vi "PicoScope3000aExampleStreamingAdvancedTrig.vi"() -> ()   [LabVIEW 2010]
doc: "This example demonstrates how to use the PicoScope Labview library to stream data from a PicoScope 5000 Series Device"
uses:
  ps3000a.dll
  ps3000aWrap.dll
  <vilib>/Waveform/DWDTOps.llb/DWDT Analog to Digital.vi
  PicoScope3000aLib/PicoScope3000aAnalogChannelSettings.ctl
  PicoScope3000aLib/PicoScope3000aDigitalChannelSettings.ctl
panel:
  in  "Pulse Width Qualifier Conditions":T1 {"Condition Logic" items=["AND", "OR", "XOR"]}
  in  "Digital Port  0":T2 {"Direction Channel 7" items=["Don't Care", "Low", "High", "Rising", "Falling"]; "Direction Channel 6" items=["Don't Care", "Low", "High", "Rising", "Falling"]; "Direction Channel 5" items=["Don't Care", "Low", "High", "Rising", "Falling"]; "Direction Channel 4" items=["Don't Care", "Low", "High", "Rising", "Falling"]; "Direction Channel 3" items=["Don't Care", "Low", "High", "Rising", "Falling"]; "Direction Channel 2" items=["Don't Care", "Low", "High", "Rising", "Falling"]; "Direction Channel 1" items=["Don't Care", "Low", "High", "Rising", "Falling"]; "Direction Channel 0" items=["Don't Care", "Low", "High", "Rising", "Falling"]}
  in  "Pulse Width Qualifier Settings":T3={"Direction"=2, "Lower Limit"=0, "Upper Limit"=0, "Pulse Width Type"=0} {"Pulse Width Type" items=["None", "Less Than", "Greater Than", "In Range", "Out of Range"]; "Direction" items=["Rising"=2, "Falling"=3]}
  in  "Auto Trigger (ms)":i32=1000
  in  "Trigger Conditions":T4 {"Condition Logic" items=["AND", "OR", "XOR"]}
  in  "Channel B Trigger Properties":T5={"thresholdUpper"=0, "thresholdUpperHysteresis"=1024, "thresholdLower"=0, "thresholdLowerHysteresis"=1024, "Threshold Mode"=0, "Direction"=2, "Available"=FALSE} {"Direction" items=["Above / Inside", "Below / Outside", "Rising / Enter", "Falling / Exit", "Rising or Falling / Enter or Exit", "Above Lower", "Below Lower", "Rising Lower", "Falling Lower", "Positive Runt", "Negative Runt"]; "Threshold Mode" items=["Level", "Window"]}
  in  "Channel A Trigger Properties":T5={"thresholdUpper"=0, "thresholdUpperHysteresis"=1024, "thresholdLower"=0, "thresholdLowerHysteresis"=1024, "Threshold Mode"=0, "Direction"=2, "Available"=FALSE} {"Direction" items=["Above / Inside", "Below / Outside", "Rising / Enter", "Falling / Exit", "Rising or Falling / Enter or Exit", "Above Lower", "Below Lower", "Rising Lower", "Falling Lower", "Positive Runt", "Negative Runt"]; "Threshold Mode" items=["Level", "Window"]}
  in  "Port 0 Settings":T6={"Enabled"=FALSE, "Logic Level"=9830} {"Logic Level" items=["1.5V TTL"=9830, "2.5V CMOS"=16383]}
  in  "Channel A Settings":T7={"Enabled"=TRUE, "Coupling"=1, "Range"=6, "Analogue Offset"=0.0, "Bandwidth Limit"=0} {"Bandwidth Limit" items=["Full", "20MHz"]; "Range" items=["10 mV", "20 mV", "50 mV", "100 mV", "200 mV", "500 mV", "1 V", "2 V", "5 V", "10 V", "20 V", "50 V ", "100 V"]; "Coupling" items=["AC", "DC"]}
  out "Analog Channels":T8(graph)
  out "Raw Sample Interval (sec)":dbl=1.0000000130088963e-06 format="%#.5p"
  out "Max ADC value":i16
  out "Chunk time":u32
  out "Elapsed time":dbl
  in  "Poll time (ms)":u32=10 min=1 max=1000 step=1
  in  "Data file":path=path "PicoScope3000aExampleStreaming ChA Data"
  out "size(s)":i32
  out "Queue depth":i32(graph)
  out "queue depth":i32
  in  "Buffer and Transfer Settings":T9={"startIndex"=0, "Samples"=1000000, "Down Sample Ratio"=1, "Down-Sample Mode"=0} {"Down-Sample Mode" items=["None"=0, "Aggregate"=1, "Decimate"=2, "Average"=4]; "Down Sample Ratio" step=1; "Samples" format="%_6p"}
  out "USB Powered":bool=TRUE
  out "USB 3.0 device on non-USB 3.0 Port":bool=TRUE
  out "TriggeredAt (In Buffer)":u32 format="%#.6p"
  out "TriggeredAt (Total samples)":u32 format="%#.6p"
  in  "Acquisition Settings":T10={"Auto Stop"=TRUE, "Desired Sample Interval"=1, "Pre-trigger Samples"=500000, "Post-trigger Samples"=500000, "Down-Sample Ratio"=1, "Down-Sample Mode"=0, "Time Units"=3} {"Time Units" items=["Nanoseconds (ns)"=2, "Microseconds (us)"=3, "Milliseconds (ms)"=4, "Seconds (s)"=5]; "Down-Sample Mode" items=["None"=0, "Aggregate"=1, "Decimate"=2, "Average"=4]; "Post-trigger Samples" format="%#.6p"; "Pre-trigger Samples" format="%#_6p"}
  out "Port 0":digitalwaveform(graph)={"t0"=timestamp(0 s since 1904-01-01), "dt"=1.0000000130088963e-06, "Y"={"transitions"=[], "data"=[]}}
  out "Triggered":bool
  out "DownSample Interval (sec)":dbl=1.0000000130088963e-06 format="%#.5p"
  out "Total Samples":u32 format="%#.6p"
  out "Auto Stopped":bool
  in  "Serial Number":string
  in  "Open Using Serial Number":bool
  out "Number of Samples per Capture":u32 format="%#.6p"
  in  "Apply  Settings":bool
  in  "stop":bool
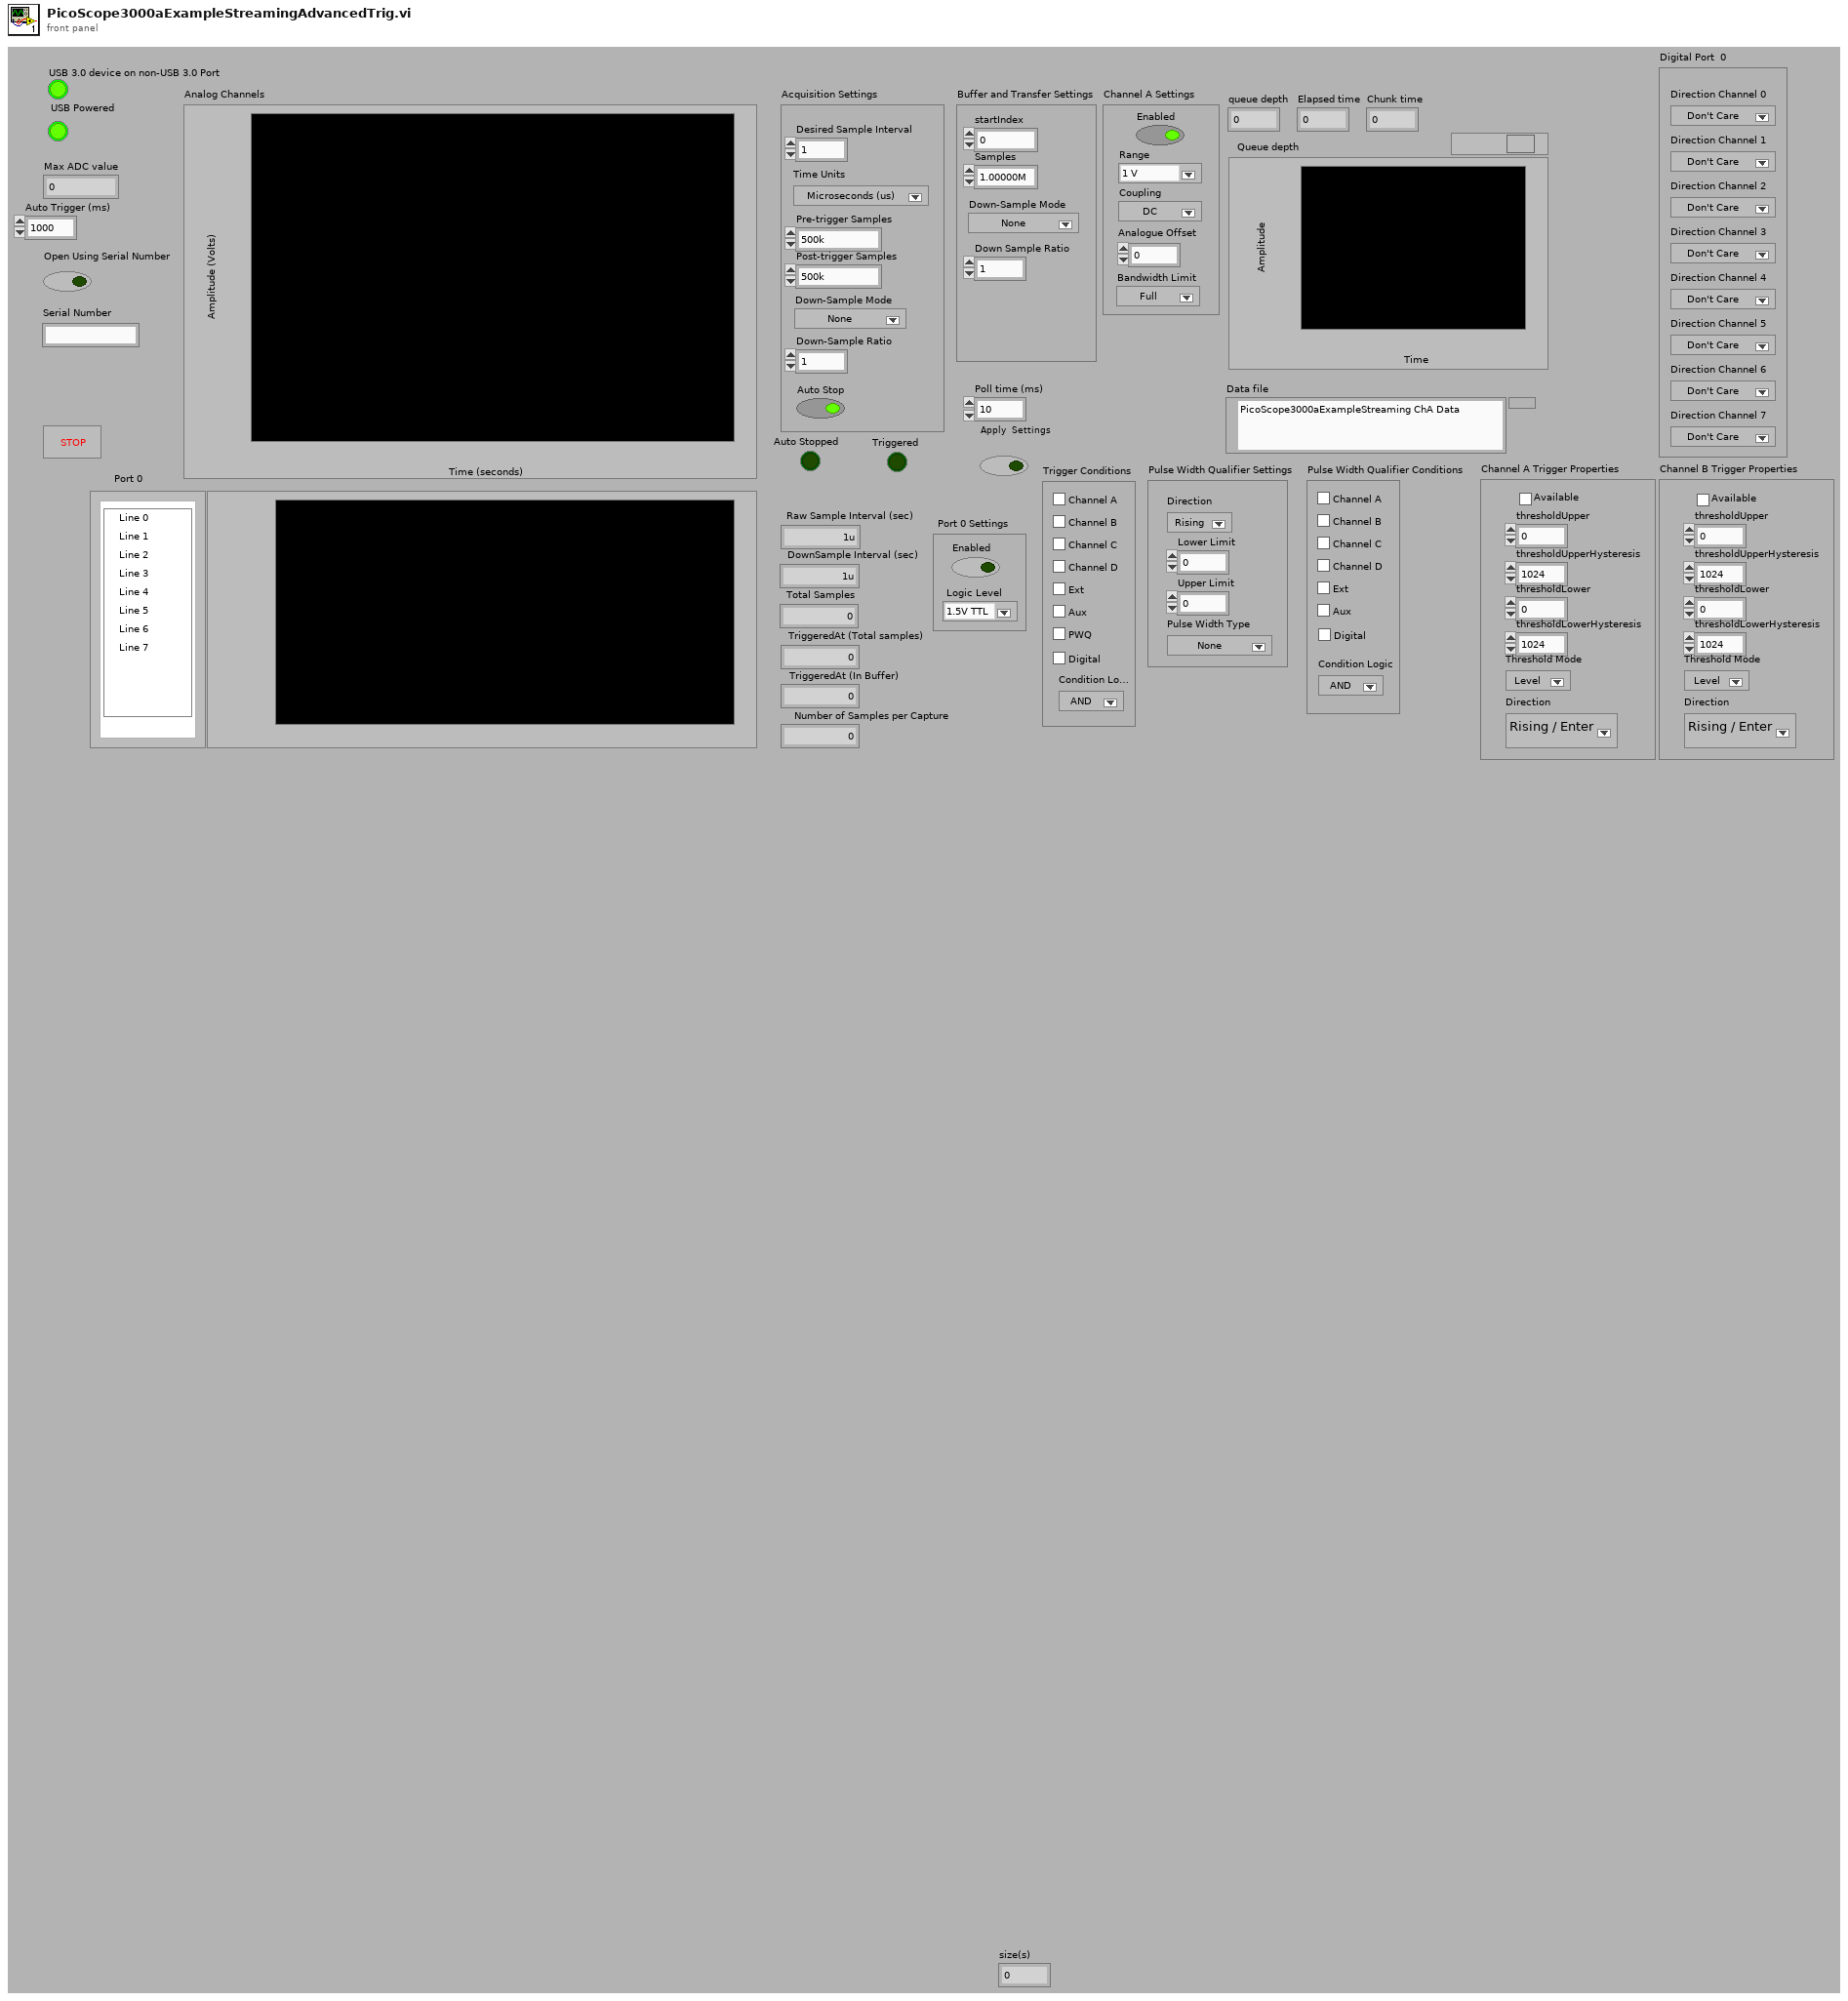
[diagram p1: front panel]
types:
  T1 = cluster{"Channel A":bool, "Channel B":bool, "Channel C":bool, "Channel D":bool, "Aux":bool, "Condition Logic":u16, "Ext":bool, "Digital":bool}
  T2 = cluster{"Direction Channel 0":u16, "Direction Channel 1":u16, "Direction Channel 2":u16, "Direction Channel 3":u16, "Direction Channel 4":u16, "Direction Channel 5":u16, "Direction Channel 6":u16, "Direction Channel 7":u16}
  T3 = cluster{"Direction":u32, "Lower Limit":u32, "Upper Limit":u32, "Pulse Width Type":u32}
  T4 = cluster{"Channel A":bool, "Channel B":bool, "Channel C":bool, "Channel D":bool, "Aux":bool, "PWQ":bool, "Condition Logic":u16, "Ext":bool, "Digital":bool}
  T5 = cluster{"thresholdUpper":i16, "thresholdUpperHysteresis":u16, "thresholdLower":i16, "thresholdLowerHysteresis":u16, "Threshold Mode":i32, "Direction":i32, "Available":bool}
  T6 = typedef "PicoScope3000aDigitalChannelSettings.ctl" = cluster{"Enabled":bool, "Logic Level":i16}
  T7 = typedef "PicoScope3000aAnalogChannelSettings.ctl" = cluster{"Enabled":bool, "Coupling":u32, "Range":u32, "Analogue Offset":sgl, "Bandwidth Limit":u32}
  T8 = cluster{i32, "DownSample Interval (sec)":dbl, "Data":dbl[]}
  T9 = cluster{"startIndex":u64, "Samples":u64, "Down Sample Ratio":u64, "Down-Sample Mode":u32}
  T10 = cluster{"Auto Stop":bool, "Desired Sample Interval":u32, "Pre-trigger Samples":u32, "Post-trigger Samples":u32, "Down-Sample Ratio":u32, "Down-Sample Mode":i32, "Time Units":u32}
  T11 = enum16{"open", "open or create", "create or replace", "create", "open (read-only)"}
  T12 = cluster{"Driver Version":string, "USB Version":string, "Hardware":string, "Variant":string, "Batch and Serial":string, "Cal Date":string, "Kernel Version":string, "Digital HW Version":string, "Analogue HW Version":string, "MSO":bool, "Number of channels":i16}
  T13 = cluster{"Channel A Buffer":i16[], "Channel B Buffer":i16[], "Channel C Buffer":i16[], "Channel D Buffer":i16[], "Channel E Buffer":i16[], "Channel F Buffer":i16[], "Channel G Buffer":i16[], "Channel H Buffer":i16[], "Port 0":i16[], "Port 1":i16[]}
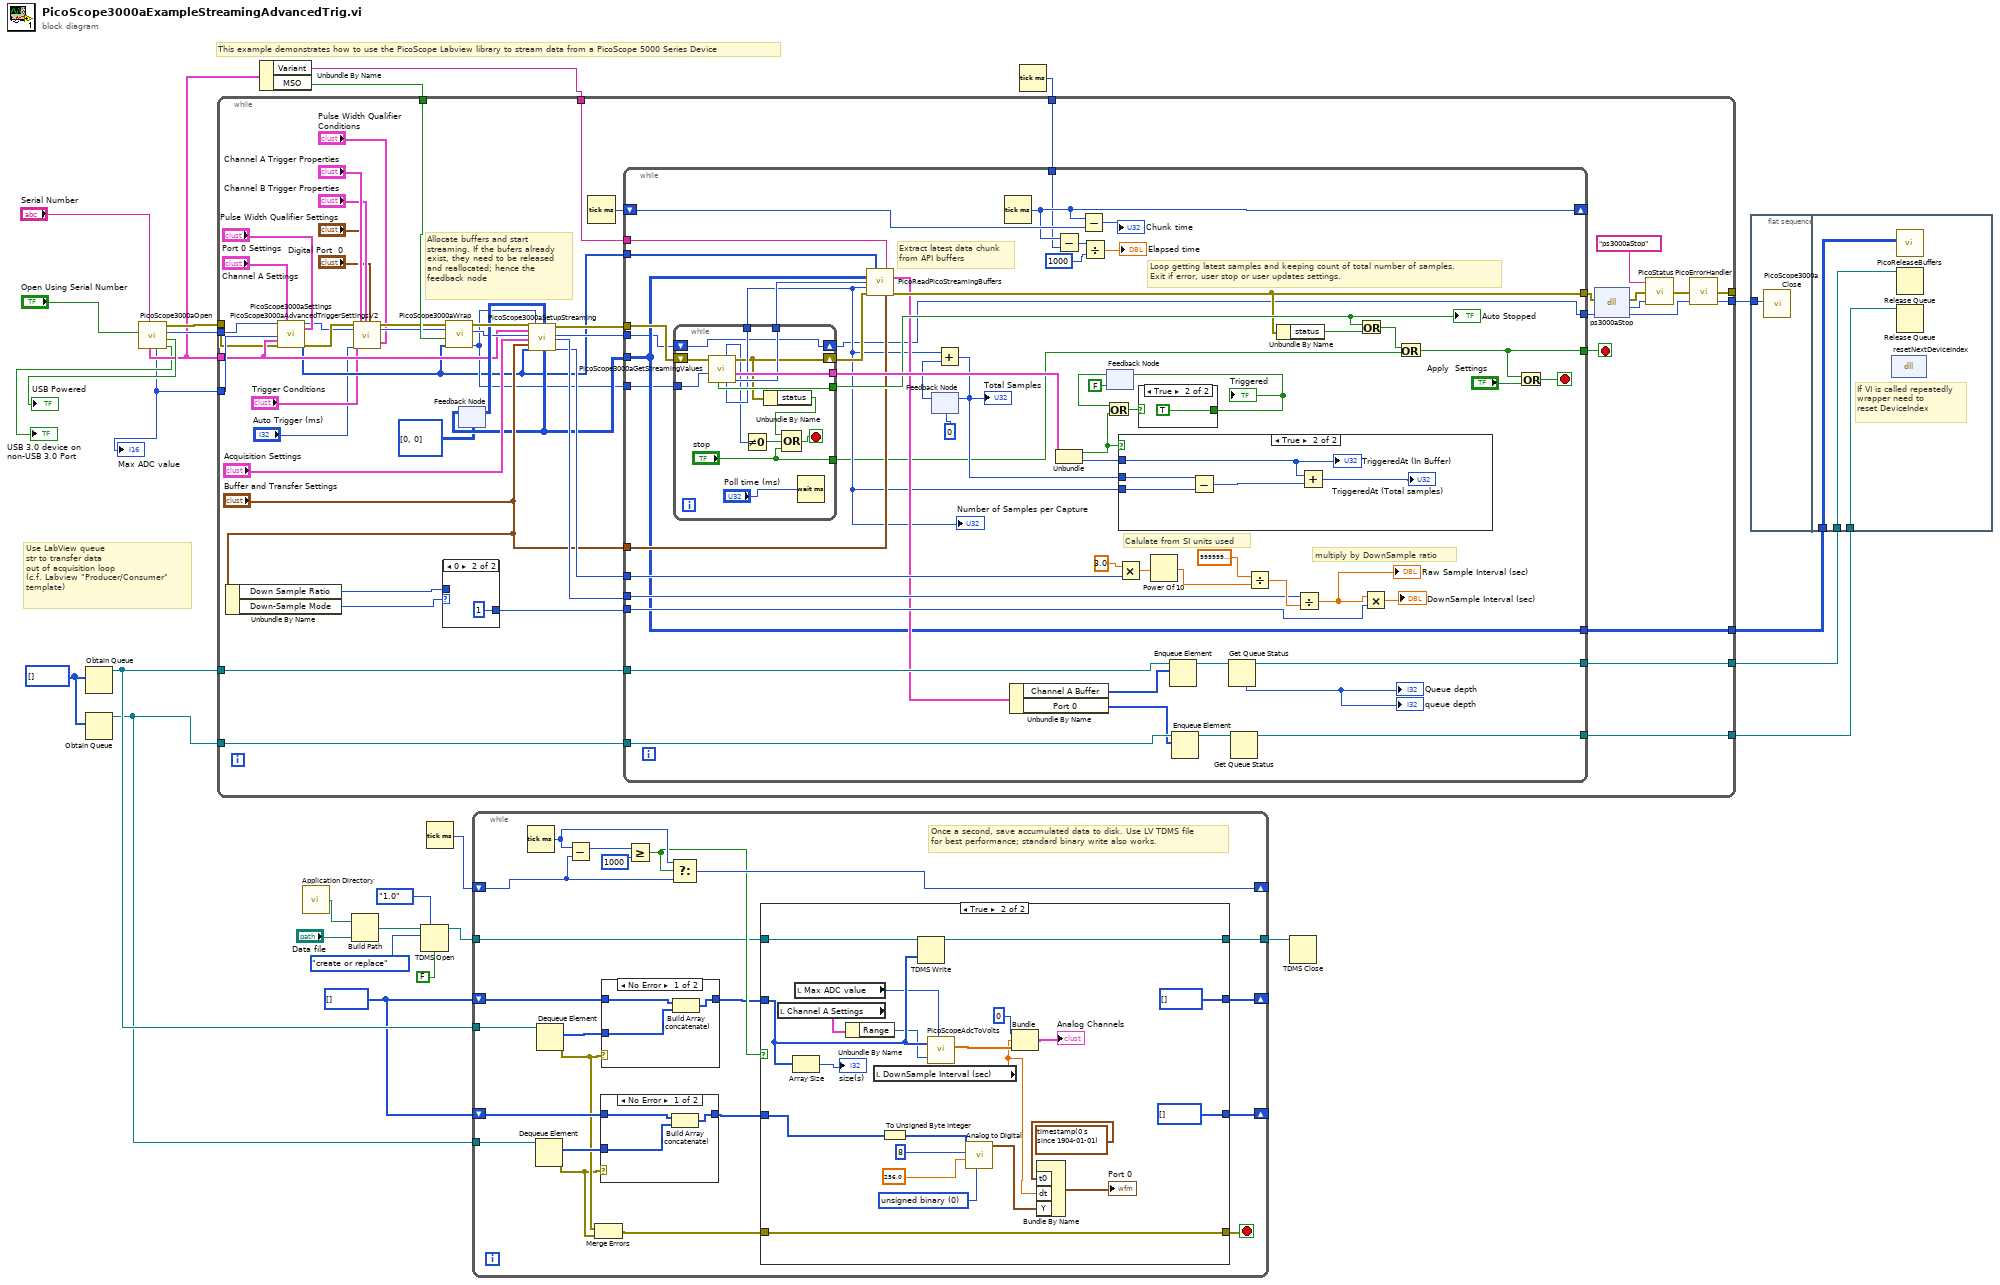
[diagram p0: block diagram]
diagram:
  w9 = i16[] [] ("History Data")
  w12 = i16[] [] ("History Data")
  # "Use LabView queue\nstr to transfer data\nout of acquisition loop\n(c.f. Labview \"Producer/Consumer\"\ntemplate)"
  # "This example demonstrates how to use the PicoScope Labview library to stream data from a PicoScope 5000 Series Device"
  n1 = Obtain Queue(element data type=w12) -> (queue out=w24:refnum<queue>)  [unwired: 4 in, 2 out]
  n2 = Obtain Queue(element data type=w12) -> (queue out=w10:refnum<queue>)  [unwired: 4 in, 2 out]
  n3 = call "PicoScope3000aOpen.vi"("Batch/Serial"="Serial Number", "Use Serial number"="Open Using Serial Number") -> ("USB 3.0 device on non-USB 3.0 Port"=→"USB 3.0 device on non-USB 3.0 Port":bool, "USB Powered"=→"USB Powered":bool, "handle"=w27:i16, "error out"=w28:errorcluster, "Max ADC value"=w1:i16, "Device Info"=w5:T12)  [unwired: 4 in]
  "Max ADC value" <- w1
  n4 = Unbundle By Name(w5) -> ("Variant"=w4:string, "MSO"=w3:bool)
  n5 = call <vilib>:"Application Directory.vi"() -> ("Application Directory"=w6:path)
  n6 = Build Path(base path=w6, name or relative path="Data file") -> (appended path=w7:path)
  n7 = TDMS Open(6:FALSE ("disable buffering? (T)"), 7:enum16{"1.0", "2.0"}."1.0" ("file format version (2.0)"), 10:T11."create or replace" ("operation (0:open)"), 11:w7) -> (3:w16:refnum<k34>)  [unwired: 2 in, 1 out]
  n8 = Tick Count (ms)() -> (millisecond timer value=w18:u32)
  n9 = while {
    tunnel: w24 -> [w49]
    shift-right: [w40] -> _
    shift-left: w9 -> [w48]
    shift-right: [w43] -> _
    shift-left: w18 -> [w44]
    tunnel: w16 -> [w39]
    tunnel: [w38] -> w15
    tunnel: w10 -> [w36]
    shift-right: [w33] -> _
    shift-left: w9 -> [w35]
    stop <- w30 stop-if-true
    # "Once a second, save accumulated data to disk. Use LV TDMS file\nfor best performance; standard binary write also works."
    n10 = Tick Count (ms)() -> (millisecond timer value=w45:u32)
    n11 = Dequeue Element(queue=w36) -> (element=w37:i16[], error out=w31:errorcluster)  [unwired: 2 in, 2 out]
    n12 = Dequeue Element(queue=w49) -> (element=w50:i16[], error out=w32:errorcluster)  [unwired: 2 in, 2 out]
    n13 = Subtract(x=w45, y=w44) -> (x-y=w47:u32)
    n14 = Merge Errors(w32, w31) -> (w29:errorcluster)
    n15 = case shown="No Error" w31 {
      tunnel: w35 -> [w53 w54]
      tunnel: [w52 w54] -> w34
      tunnel: w37 -> [w51 _]
      frame No Error {
        n16 = Build Array (concatenate)(w53, w51) -> (w52:i16[])
      }
      frame Error {
      }
    }
    n17 = case shown="No Error" w32 {
      tunnel: w48 -> [w83 w84]
      tunnel: [w82 w84] -> w41
      tunnel: w50 -> [w81 _]
      frame No Error {
        n18 = Build Array (concatenate)(w83, w81) -> (w82:i16[])
      }
      frame Error {
      }
    }
    n19 = Greater Or Equal?(x=w47, y=u32 1000) -> (x >= y?=w42:bool)
    n20 = Select(t=w45, s=w42, f=w44) -> (s? t:f=w43:u32)
    n21 = case shown="True" w42 {
      tunnel: w41 -> [w58 w76]
      tunnel: [w58 i16[] [] ("History Data")] -> w40
      tunnel: w39 -> [w57 w78]
      tunnel: [w57 w77] -> w38
      tunnel: w34 -> [w56 w63]
      tunnel: [w56 i16[] [] ("History Data")] -> w33
      tunnel: [w55 w59] -> w30
      tunnel: w29 -> [w55 w59]
      frame False {
      }
      frame True {
        w69 = u16 0 items=["unsigned binary", "offset binary", "2's complement"] ("data format (offset binary)")
        n22 = local read "Channel A Settings"() -> (w60:T7)
        n23 = Array Size(array=w76) -> (size(s)=→"size(s)":i32)
        n24 = local read "Max ADC value"() -> (w72:i16)
        n25 = Unbundle By Name(w60) -> ("Range"=w75:u32)
        n26 = local read "DownSample Interval (sec)"() -> (w64:dbl)
        n27 = To Unsigned Byte Integer(number=w63) -> (unsigned 8bit integer=w68:u8[])
        n28 = TDMS Write(0:w78, 9:w76) -> (4:w77:refnum<k34>)  [unwired: 4 in, 3 out]
        n29 = call "PicoScopeAdcToVolts.vi"("Max_adc"=w72, "Range Index"=w75, "Data"=w76) -> ("Data"=w73:dbl[])
        n30 = call-poly <vilib>:"Analog to Digital.vi"("data format (offset binary)"=w69, "full-scale range (pk-pk)"=256.0, "resolution (16 bit)"=8, "analog waveform"=w68) -> ("digital waveform"=w65:digitalwaveform)  [unwired: 4 in, 3 out]
        n31 = Bundle(0, "DownSample Interval (sec)"=w64, "Data"=w73) -> (→"Analog Channels":T8)  [unwired: 1 in]
        n32 = Bundle By Name("t0"=timestamp(0 s since 1904-01-01), "dt"=w64, "Y"=w65) -> (→"Port 0":digitalwaveform)  [unwired: 1 in]
      }
    }
  }
  n33 = Tick Count (ms)() -> (millisecond timer value=w23:u32)
  n34 = while {
    tunnel: [w131] -> w22
    tunnel: w28 -> [w98]
    tunnel: w27 -> [w97]
    tunnel: w5 -> [w100]
    tunnel: w1 -> [w103]
    tunnel: [w117] -> w20
    tunnel: w24 -> [w116]
    tunnel: [w115] -> w21
    tunnel: [w113] -> _
    tunnel: w23 -> [w111]
    tunnel: [w108] -> w11
    tunnel: w10 -> [w107]
    tunnel: w4 -> [w106]
    tunnel: w3 -> [w104]
    stop <- w135 stop-if-true
    # "Allocate buffers and start\nstreaming. If the bufers already\nexist, they need to be released\nand reallocated; hence the\nfeedback node"
    n35 = Unbundle By Name("Buffer and Transfer Settings") -> ("Down Sample Ratio"=w120:u64, "Down-Sample Mode"=w122:u32)
    n36 = call "PicoScope3000aSettings.vi"("handle in"=w97, "Channel A Settings"="Channel A Settings", "Port 0 Settings"="Port 0 Settings", "Max_adc"=w103, "Device Info"=w100, "error in"=w98) -> ("handle out"=w94:i16, "Enabled Array"=w96:i16[], "error out"=w95:errorcluster)  [unwired: 7 in]
    n37 = call "PicoScope3000aAdvancedTriggerSettingsV2.vi"("error in"=w95, "handle in"=w94, "Trigger Conditions"="Trigger Conditions", "Auto Trigger (ms)"="Auto Trigger (ms)", "Channel A Trigger Properties"="Channel A Trigger Properties", "Channel B Trigger Properties"="Channel B Trigger Properties", "Digital Port  0"="Digital Port  0", "Pulse Width Qualifier Conditions"="Pulse Width Qualifier Conditions", "Pulse Width Qualifier Settings"="Pulse Width Qualifier Settings") -> ("error out"=w93:errorcluster, "handle out"=w92:i16)  [unwired: 9 in]
    n38 = case shown="0" w122 {
      tunnel: [w136 u32 1 ("Down-Sample Ratio")] -> w121
      tunnel: w120 -> [w136 _]
      frame Default {
      }
      frame 0 {
      }
    }
    n39 = call "PicoScope3000aWrap.vi"("Enabled Array"=w96, "MSO Device?"=w104, "handle in"=w92, "error in (no error)"=w93) -> ("deviceIndex"=w99:u16, "handle out"=w101:i16, "error out"=w126:errorcluster)  [unwired: 1 in]
    n40 = feedback #1(u64[][] [[0], [0]] ("Pointer array")) -> (w114:u64[][])
    n41 = call "PicoScope3000aSetupStreaming.vi"("error in"=w126, "Device Info"=w100, "handle in"=w101, "Acquisition Settings"="Acquisition Settings", "Buffer and Transfer Settings"="Buffer and Transfer Settings", "enabled array"=w96, "deviceIndex"=w99, "Pointers In"=w114) -> ("Pointer array"=w110:u64[][], "error out"=w133:errorcluster, "handle out"=w134:i16, "Sample Interval"=w125:u32, "sampleIntervalTimeUnits"=w124:u32)  [unwired: 7 in]
    n42 = feedback-in #1(w110) -> ()
    n43 = Tick Count (ms)() -> (millisecond timer value=w112:u32)
    n44 = while {
      tunnel: [w138] -> w132
      tunnel: [w192] -> w135
      tunnel: w134 -> [w139]
      tunnel: w133 -> [w168]
      tunnel: w125 -> [w171]
      tunnel: w124 -> [w179]
      tunnel: [w165] -> w123
      tunnel: w121 -> [w169]
      tunnel: "Buffer and Transfer Settings" -> [w167]
      tunnel: w96 -> [w164]
      tunnel: [w162] -> w117
      tunnel: w116 -> [w160]
      tunnel: w110 -> [w158]
      tunnel: [w158] -> w115
      shift-right: [w153] -> _
      shift-left: w112 -> [w154]
      tunnel: w111 -> [w152]
      tunnel: w106 -> [w147]
      tunnel: [w144] -> w108
      tunnel: w107 -> [w143]
      tunnel: w99 -> [w140]
      stop <- w191 stop-if-true
      # "Loop getting latest samples and keeping count of total number of samples. \nExit if error, user stop or user updates settings."
      # "Extract latest data chunk\nfrom API buffers"
      # "Calulate from SI units used"
      # "multiply by DownSample ratio"
      n45 = while {
        tunnel: [w207] -> w190
        tunnel: [w206] -> w187
        tunnel: [w204] -> w149
        tunnel: [w203] -> w148
        shift-right: [w195] -> w138
        shift-left: w139 -> [w195]
        shift-right: [w202] -> w166
        shift-left: w168 -> [w205]
        tunnel: ["stop"] -> w141
        tunnel: w140 -> [w194]
        stop <- w197 stop-if-true
        n46 = call "PicoScope3000aGetStreamingValues.vi"("deviceIndex"=w194, "error in"=w205) -> ("Start Index"=w204:u32, "Trigger"=w207:cluster{bool, "triggeredAt (Total samples)":u32}, "error out"=w202:errorcluster, "Number of Samples"=w203:i32, "ready"=w200:i16, "Auto Stopped"=w206:bool)  [unwired: 4 in]
        n47 = Not Equal To 0?(x=w200) -> (x != 0?=w198:bool)
        n48 = Unbundle By Name(w202) -> ("status"=w199:bool)
        n49 = Compound Arithmetic op=OR(w199, w198, "stop") -> (w197:bool)
        n50 = Wait (ms)(milliseconds to wait="Poll time (ms)") -> ()  [unwired: 1 out]
      }
      "Number of Samples per Capture" <- w148
      "Auto Stopped" <- w187
      n51 = call "PicoReadPicoStreamingBuffers.vi"("enabled array"=w164, "Buffer and Transfer Settings"=w167, "Variant"=w147, "Pointer array"=w158, "Offset Index"=w149, "Number of Samples"=w148, "error in (no error)"=w166) -> ("Buffers (Max or non-aggregated)"=w159:T13, "error out"=w165:errorcluster)  [unwired: 6 in, 1 out]
      n52 = feedback #2(u32 0) -> (w183:u32)
      n53 = Add(x=w148, y=w183) -> (x+y=w175:u32)
      "Total Samples" <- w175
      n54 = feedback-in #2(w175) -> ()
      n55 = Tick Count (ms)() -> (millisecond timer value=w153:u32)
      n56 = Unbundle By Name(w159) -> ("Channel A Buffer"=w150:i16[], "Port 0"=w142:i16[])
      n57 = Subtract(x=w153, y=w152) -> (x-y=w157:u32)
      n58 = Unbundle(w190) -> (w173:bool, "triggeredAt (Total samples)"=w172:u32)
      n59 = Subtract(x=w153, y=w154) -> (x-y=→"Chunk time":u32)
      n60 = Divide(x=w157, y=u32 1000) -> (x/y=→"Elapsed time":dbl)
      n61 = feedback #3(FALSE) -> (w185:bool)
      n62 = Or(x=w185, y=w173) -> (x .or. y?=w176:bool)
      n63 = Multiply(x=3.0, y=w179) -> (x*y=w177:dbl)
      n64 = case shown="True" w173 {
        tunnel: w148 -> [_ w208]
        tunnel: w175 -> [_ w212]
        tunnel: w172 -> [_ w210]
        frame False {
        }
        frame True {
          n65 = Subtract(x=w212, y=w208) -> (x-y=w211:u32)
          n66 = Add(x=w210, y=w211) -> (x+y=→"TriggeredAt (Total samples)":u32)
          "TriggeredAt (In Buffer)" <- w210
        }
      }
      n67 = case shown="True" w176 {
        selector: w176 -> [w213 _]
        tunnel: [w213 TRUE] -> w174
        frame False {
        }
        frame True {
        }
      }
      "Triggered" <- w174
      n68 = feedback-in #3(w174) -> ()
      n69 = Power Of 10(x=w177) -> (10^x=w178:dbl)
      n70 = Enqueue Element(queue=w160, element=w150) -> (queue out=w161:refnum<queue>)  [unwired: 2 in, 2 out]
      n71 = Enqueue Element(queue=w143, element=w142) -> (queue out=w145:refnum<queue>)  [unwired: 2 in, 2 out]
      n72 = Get Queue Status(queue=w161) -> (queue out=w162:refnum<queue>, # elements in queue=→"queue depth" →"Queue depth":i32)  [unwired: 2 in, 6 out]
      n73 = Get Queue Status(queue=w145) -> (queue out=w144:refnum<queue>)  [unwired: 2 in, 7 out]
      n74 = Divide(x=sgl 1000000000000000.0 ("y"), y=w178) -> (x/y=w180:dbl)
      n75 = Unbundle By Name(w165) -> ("status"=w189:bool)
      n76 = Divide(x=w171, y=w180) -> (x/y=w146:dbl)
      "Raw Sample Interval (sec)" <- w146
      n77 = Or(x=w187, y=w189) -> (x .or. y?=w188:bool)
      n78 = Multiply(x=w146, y=w169) -> (x*y=→"DownSample Interval (sec)":dbl)
      n79 = Or(x=w188, y=w141) -> (x .or. y?=w192:bool)
      n80 = Or(x=w192, y="Apply  Settings") -> (x .or. y?=w191:bool)
    }
    n81 = dll-call lib="ps3000a.dll" fn="ps3000aStop"(error in=w123, "handle"=w132) -> (error out=w129:errorcluster, "PICO_STATUS"=w130:u32, "handle"=w131:i16)  [unwired: 2 in, 1 out]
    n82 = call "PicoStatus.vi"("PICO STATUS"=w130, "error in"=w129, "source"="ps3000aStop") -> ("error out"=w128:errorcluster)
    n83 = call "PicoErrorHandler.vi"("error in"=w128) -> ("error out"=w113:errorcluster)
  }
  n84 = TDMS Close(11:w15) -> ()  [unwired: 1 in, 2 out]
  n85 = flat-sequence {
    tunnel: w22 -> [w215]
    tunnel: w21 -> [w218]
    tunnel: w20 -> [w217]
    tunnel: w11 -> [w216]
    frame #0 {
      n86 = call "PicoScope3000aClose.vi"("handle"=w215) -> ()
    }
    frame #1 {
      # "If VI is called repeatedly\nwrapper need to\nreset DeviceIndex"
      n87 = dll-call lib="ps3000aWrap.dll" fn="resetNextDeviceIndex"() -> ()  [unwired: 4 in, 2 out]
      n88 = call "PicoReleaseBuffers.vi"("Pointer array"=w218) -> ()  [unwired: 10 in, 1 out]
      n89 = Release Queue(queue=w217) -> ()  [unwired: 2 in, 3 out]
      n90 = Release Queue(queue=w216) -> ()  [unwired: 2 in, 3 out]
    }
  }
